vi "CIF_Iceoryx Channel Performance Test.vi"() -> ()   [LabVIEW 2021]
uses:
  Double/CIF_Iceoryx_Chn_Double.lvclass
  D:/dev/Packages/CIF_Channels_Core/src/Iceorxy_Channels/CIF_Iceoryx_BB/CIF_Iceoryx_BB.lvclass
  D:/dev/Packages/CIF_Channels_Core/src/CIFChannels/CIFChannels.lvclass
  ChannelCommon/typedef/Direction.ctl
  <vilib>/CIF Foundation/CIF Iceoryx/typedef/Topic Full Names.ctl
  <vilib>/Platform/TimedLoop/XDataNode/timing_clust.ctl
  <vilib>/Platform/TimedLoop/XDataNode/nitl_modes.ctl
  <vilib>/Platform/TimedLoop/XDataNode/wakeup.ctl
  ChannelCommon/typedef/New FIFO Instance Response.ctl
  CIFChannels/CIFChannels.lvclass/CIFChannels.ctl
  CIF_Iceoryx_BB/CIF_Iceoryx_BB.lvclass/CIF_Iceoryx_BB.ctl
  Double/CIF_Iceoryx_Chn_Double.lvclass/CIF_Iceoryx_Chn_Double.ctl
  53e91fa4-a651-41f7-b02c-832fa8f08f6c.vi
  a00a81b1-57b6-4108-a755-745f4eb81d77.vi
  b62546a3-05e7-4285-b37f-cb0405f50769.vi
  14a2fe34-1335-4f7a-a7a9-124bb301578e.vi
  14bdf759-0034-46fe-882d-46e8766a29d9.vi
  ec66e212-9a84-4060-a812-2933347e74f4.vi
  182f4b0c-1596-45c4-9e4a-6a0b9b3960fd.vi
  <vilib>/CIF Foundation/CIF Iceoryx/SubVIs/Get Path.vi
  <vilib>/CIF Foundation/CIF Iceoryx/SubVIs/Convert Error.vi
  53e91fa4-a651-41f7-b02c-832fa8f08f6c.vi/f164bb55-fadc-406a-97d8-e3295a396b46.vi
  <vilib>/CIF Foundation/CIF Iceoryx/SubVIs/Add Error.vi
  <vilib>/CIF Foundation/CIF Iceoryx/Refnum/BB from Refnum.vi
  <vilib>/CIF Foundation/CIF Iceoryx/Refnum/BB Writer to Refnum.vi
  a00a81b1-57b6-4108-a755-745f4eb81d77.vi/15451e88-64ef-462d-9cc0-58968935b893.vi
  <vilib>/CIF Foundation/CIF Iceoryx/Refnum/BB Writer from Refnum.vi
  <vilib>/CIF Foundation/CIF Iceoryx/Refnum/BB Reader from Refnum.vi
  Double/Core/Read Double Direct.vi/e9c5801a-3ed8-4028-afd6-45613173f8eb.vi
  CIF_Iceoryx_BB/Accessors/Read Reader Reference.vi
  CIFChannels/Accessors/Read Tag Forced.vi
  CIFChannels/Accessors/Read Channel State.vi
  CIFChannels/Accessors/Read Direction.vi
  Double/Core/Write Double Direct.vi/36393718-afdf-41a6-b430-da9823bc1f33.vi
  CIF_Iceoryx_BB/Accessors/Read Writer Reference.vi
  <vilib>/Utility/error.llb/Trim Whitespace.vi
  <vilib>/CIF Foundation/CIF Iceoryx/SubVIs/Add Error Core.vi
  <vilib>/CIF Foundation/CIF Utilities/DataTypes/Utilities/Get Element Info of Variant.vi
  <vilib>/CIF Foundation/CIF Iceoryx/SubVIs/Get Type String.vi
  <vilib>/CIF Foundation/CIF Utilities/DataTypes/Utilities/Get JSON Descriptor of Variant.vi
  <vilib>/CIF Foundation/CIF Iceoryx/SubVIs/Convert Error Core.vi
  <vilib>/CIF Foundation/CIF Iceoryx/Blackboard/Create Abstracted Reader.vi
  <vilib>/Platform/TimedLoop/XDataNode/XDataNode.xnode
  <vilib>/Platform/TimedLoop/XDataNode/XDNodeRunTimeDep.lvlib
  <vilib>/CIF Foundation/CIF Iceoryx/Iceoryx.lvlib
  ChannelCommon/ChannelCommon.lvlib
  CIF_Iceoryx_BB/CIF_Iceoryx_BB.lvclass
  CIFChannels/CIFChannels.lvclass
panel:
  out "avg dbl channel write":dbl
  out "max dbl channel write":dbl
  out "avg dbl channel dd":dbl
  out "max dbl channel dd":dbl
  in  "Stop":bool
  out "avg dbl channel":dbl
  out "max dbl channel":dbl
  out "avg raw channel":dbl
  out "max raw channel":dbl
  out "pass":bool
  out "error out":errorcluster
  # "This test should be run on RT.  It stresses the communications by constantly creating resource contraints with the low priority sender and the high priority loop. On Windows the priority of the loops cannot be set."
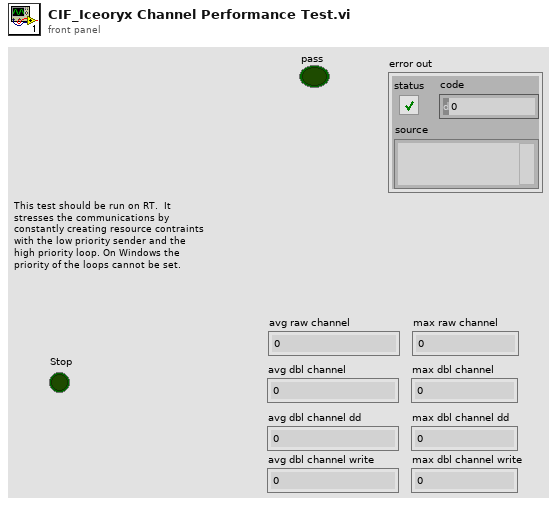
[diagram p1: front panel]
types:
  T1 = typedef "ChannelCommon.lvlib/Direction.ctl" = enum8{"Publisher", "Subscriber"}
  T2 = typedef "Iceoryx.lvlib/Topic Full Names.ctl" = cluster{"BlackBoard":string, "Topic":string, "Type Override":string}
  T3 = typedef "XDNodeRunTimeDep.lvlib/timing_clust.ctl" = cluster{"Expected End [f-1]":u64, "Actual End [f-1]":u64, "Finished Late? [f-1]":bool, "Expected End [i-1]":u64, "Actual End [i-1]":u64, "Finished Late? [i-1]":bool, "Expected Start [i]":u64, "Actual Start [i]":u64, "Expected Start [f]":u64, "Actual Start [f]":u64, "Source Name":string, "Structure Name":string, "Period":i64, "Deadline":i64, "Offset":i64, "Start":i64, "Priority":i32, "Timeout":i32, "Mode":T4, "Wakeup Reason":T5, "Error":errorcluster, "Source Type":string, "Secondary Source Type":string, "Global End Time":u64, "Global Start Time":u64, "Frame Duration":u64, "Iteration Duration":u64, "Assigned CPU":i32, "I/O Scan Engine Mode":u32}
  T4 = typedef "XDNodeRunTimeDep.lvlib/nitl_modes.ctl" = enum32{"No Change", "Process missed periods, maintain original phase", "Discard missed periods, maintain original phase", "Process missed periods, ignore original phase", "Discard missed periods, ignore original phase"}
  T5 = typedef "XDNodeRunTimeDep.lvlib/wakeup.ctl" = enum32{"Normal", "Aborted", "Asynchronous wakeup", "Timing source error", "Timed loop error", "Timeout"}
  T6 = typedef "ChannelCommon.lvlib/New FIFO Instance Response.ctl" = cluster{"Publisher":string, "Custom Data":u8[]}
  T7 = typedef "Iceoryx.lvlib/BB Refnum.ctl" = cluster{"refnum":u64, "BB":enum8{"bb"}}
  T8 = typedef "Iceoryx.lvlib/BB Writer Refnum.ctl" = cluster{"refnum":u64, "BB Writer":enum8{"bb_writer"}}
  T9 = typedef "Iceoryx.lvlib/BB Reader Refnum.ctl" = cluster{"refnum":u64, "BB Reader":enum8{"bb_reader"}}
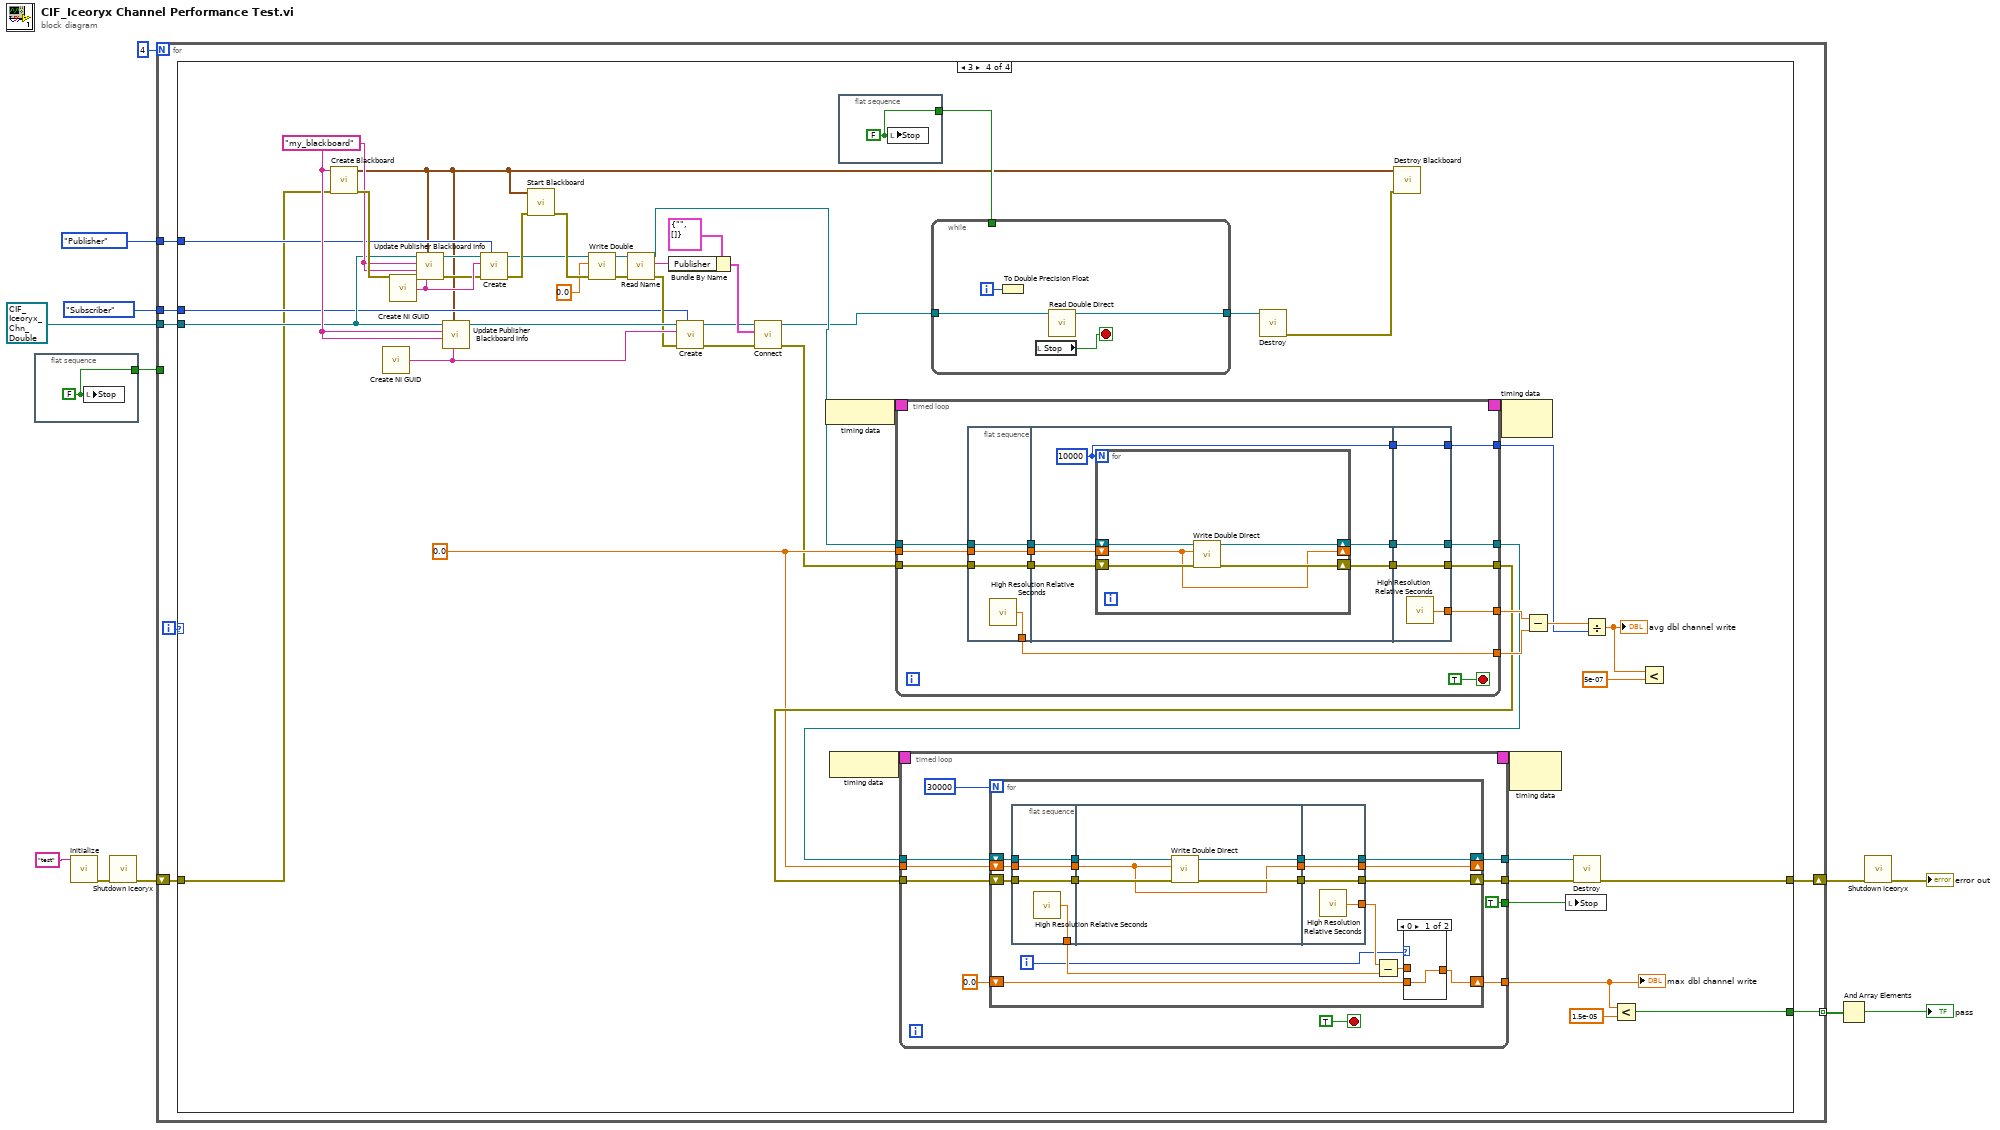
[diagram p0: block diagram]
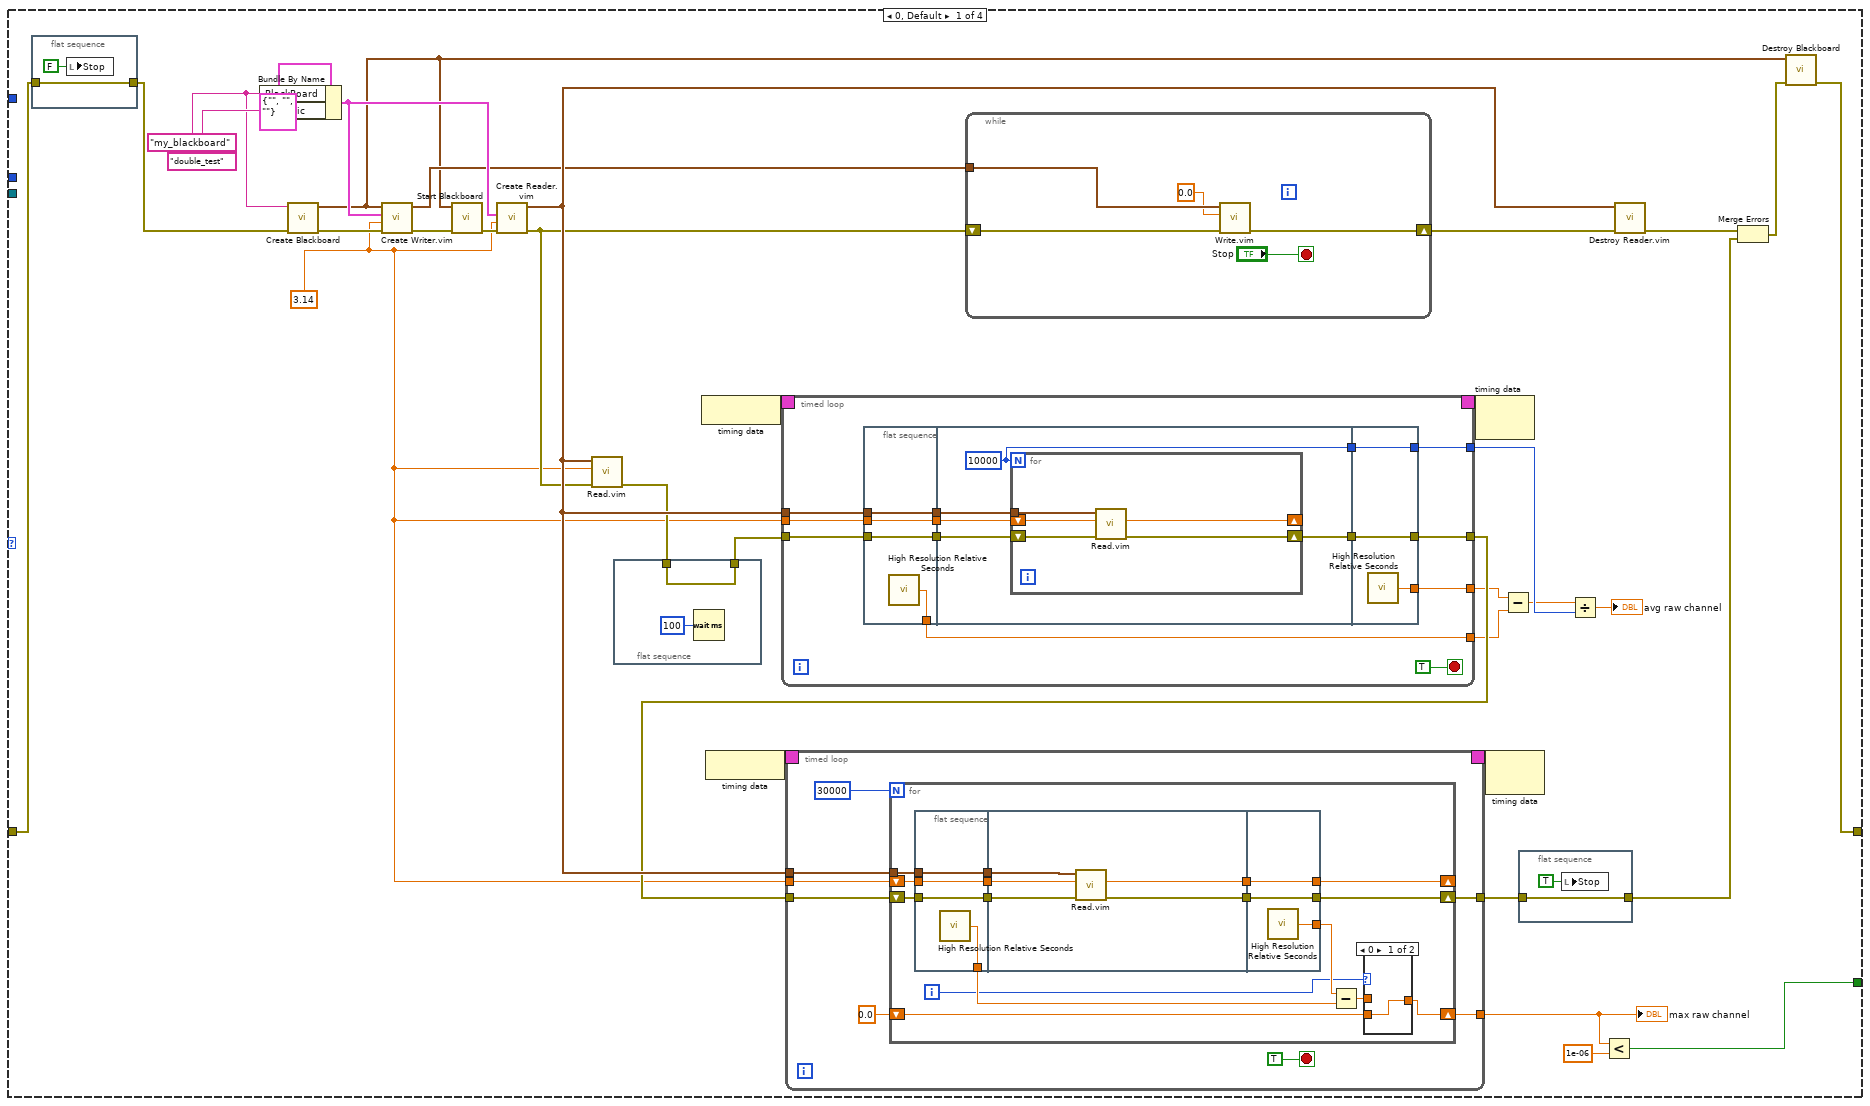
[diagram p2: hidden frame]
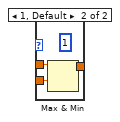
[diagram p3: hidden frame]
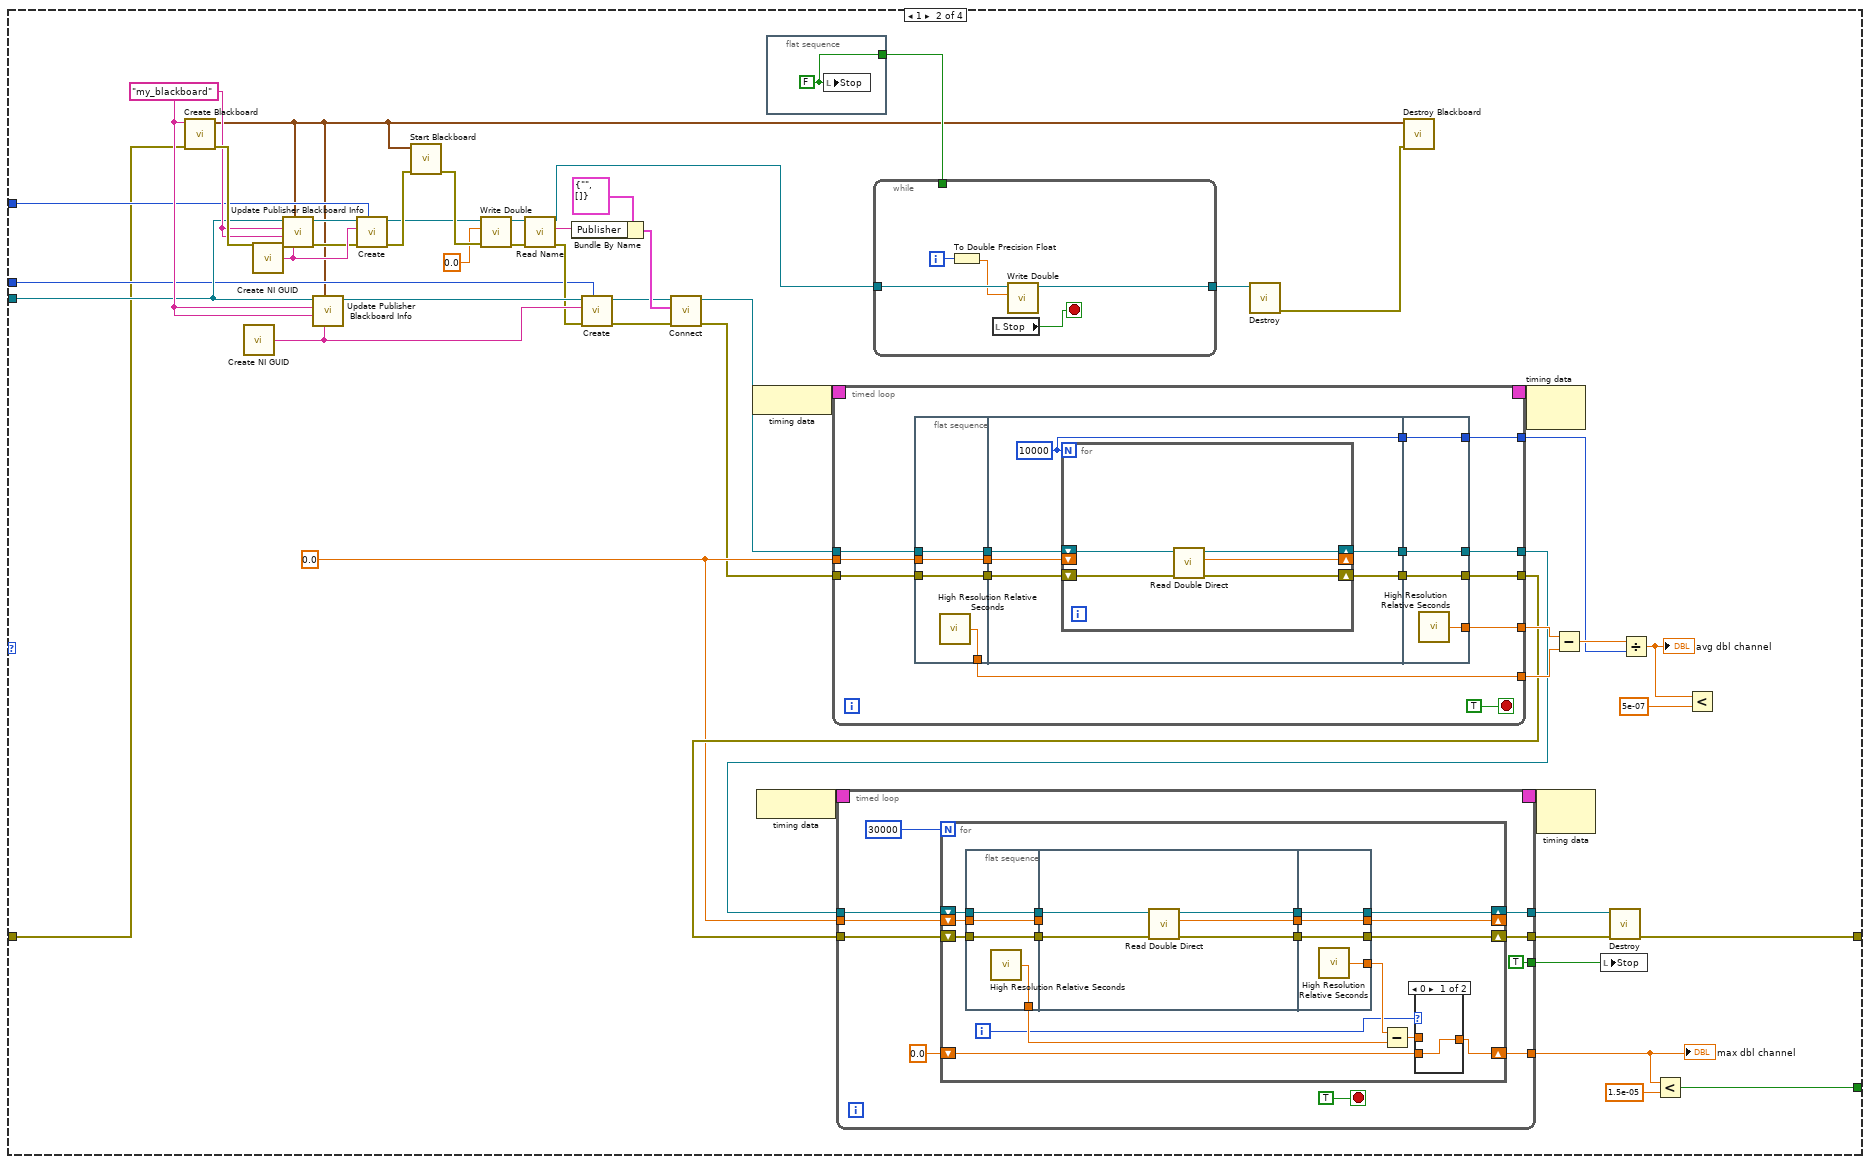
[diagram p4: hidden frame]
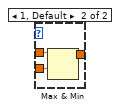
[diagram p5: hidden frame]
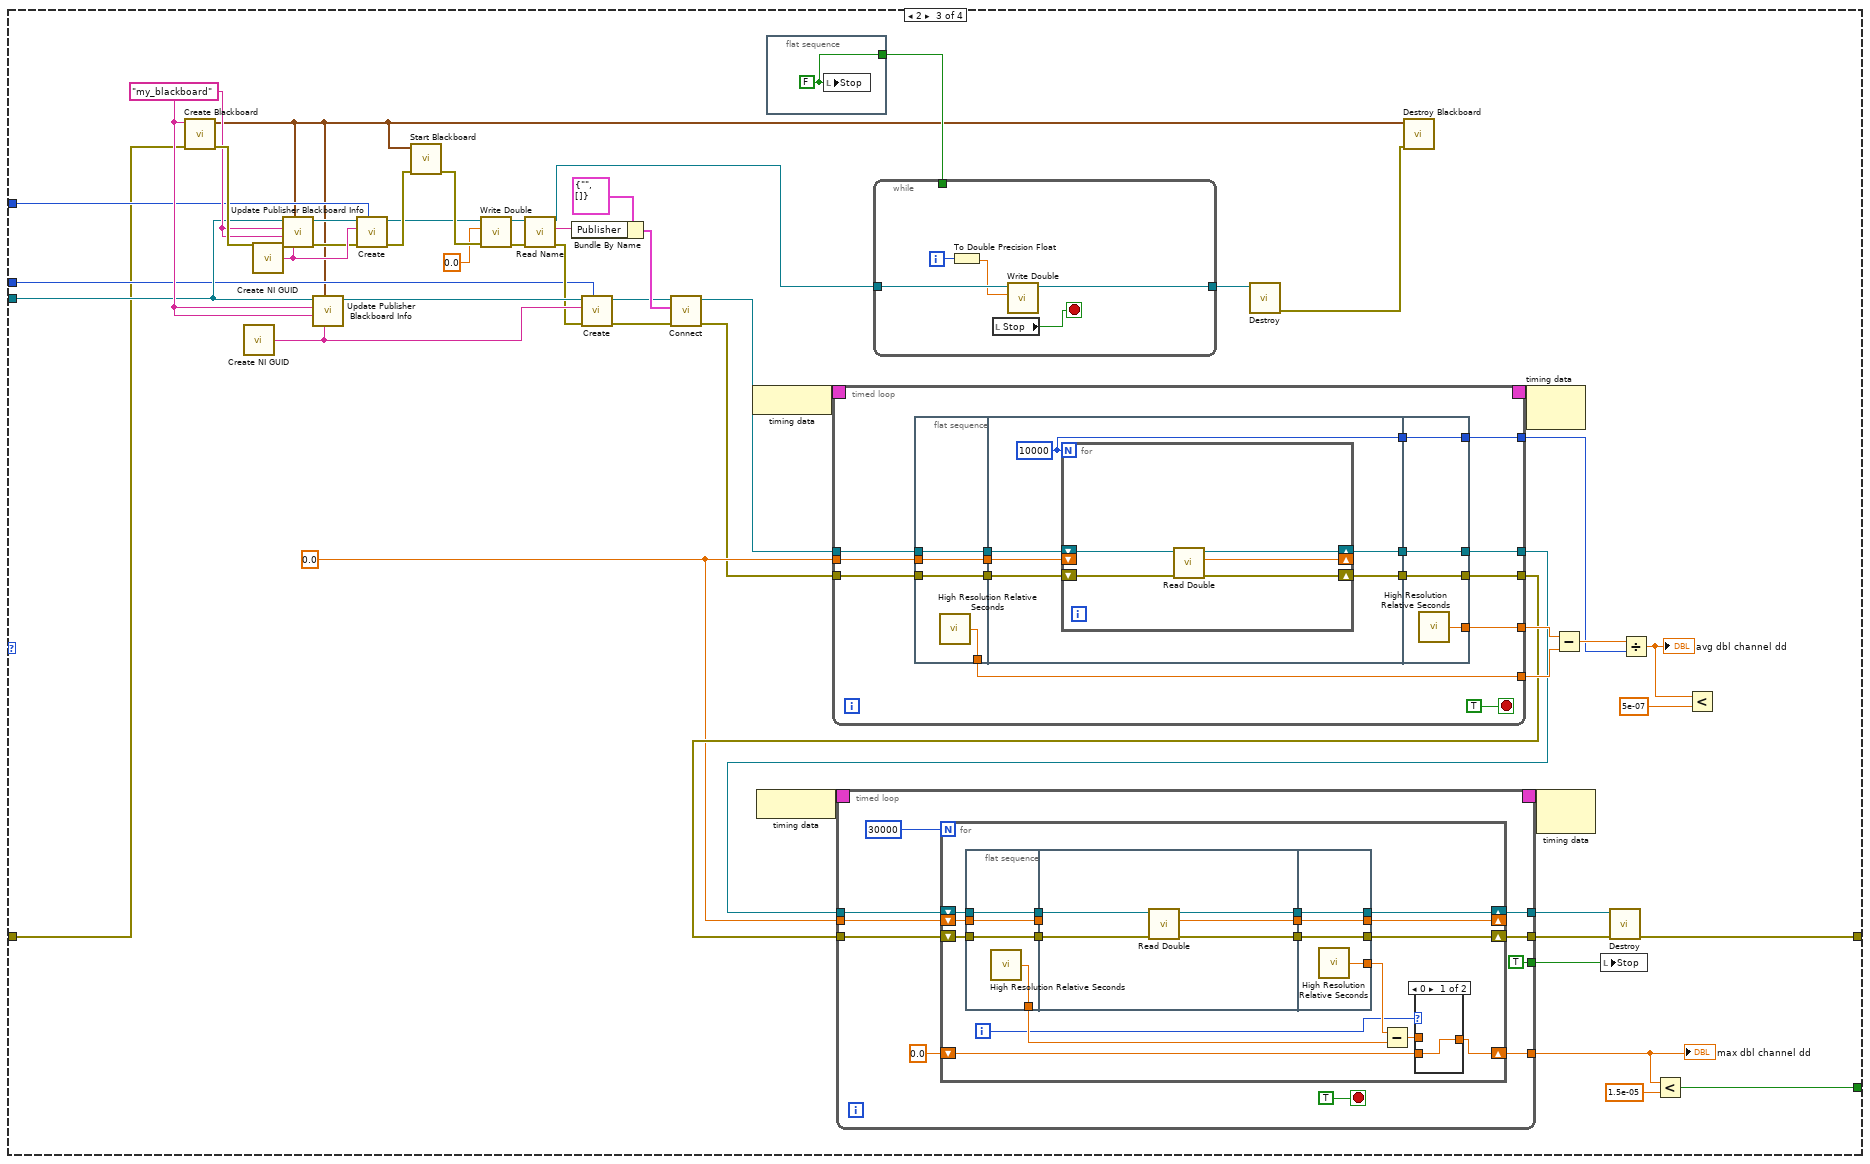
[diagram p6: hidden frame]
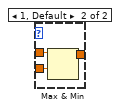
[diagram p7: hidden frame]
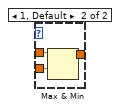
[diagram p8: hidden frame]
diagram:
  n1 = flat-sequence {
    tunnel: [w13] -> w8
    frame #0 {
      w13 = FALSE ("Stop")
      n2 = local write "Stop"(w13) -> ()
    }
  }
  n3 = call <vilib>:"Initialize.vi"("Node name"="test") -> ("error out"=w4:errorcluster)  [unwired: 10 in]
  n4 = call <vilib>:"Shutdown Iceoryx.vi"("error in (no error)"=w4) -> ("error out"=w3:errorcluster)  [unwired: 10 in]
  n5 = for {
    N: 4 -> [_]
    tunnel: [w20] -> w11 mode=indexing
    shift-right: [w19] -> w2
    shift-left: w3 -> [w17]
    tunnel: refnum<class "CIF_Iceoryx_Chn_Double.lvclass"> refnum ("CIF_CIPC_Chn_Double.lvclass") -> [w16]
    tunnel: w8 -> [_]
    tunnel: Direction."Publisher" ("Direction") -> [w15]
    tunnel: Direction."Subscriber" ("Direction") -> [w14]
    i -> [w18]
    n6 = case shown="3" w18 {
      tunnel: [w25 w180 w323 w466] -> w20
      tunnel: [w24 w176 w319 w462] -> w19
      tunnel: w17 -> [w30 w147 w290 w434]
      tunnel: w16 -> [_ w154 w297 w440]
      tunnel: w15 -> [_ w153 w296 w439]
      tunnel: w14 -> [_ w152 w295 w438]
      frame 0, Default {
        w22 = "my_blackboard" ("Blackboard name")
        w23 = 3.14 ("Data")
        n7 = flat-sequence {
          tunnel: w30 -> [w62]
          tunnel: [w62] -> w48
          frame #0 {
            n8 = local write "Stop"(FALSE ("stop")) -> ()
          }
        }
        n9 = Bundle By Name(cluster=T2 {"BlackBoard"="", "Topic"="", "Type Override"=""} ("Topic Full Names"), "BlackBoard"=w22, "Topic"="double_test" ("topic")) -> (w45:T2)
        n10 = call <vilib>:"Create Blackboard.vi"("error in (no error)"=w48, "Blackboard name"=w22) -> ("error out"=w38:errorcluster, "Blackboard Reference"=w40:T7)  [unwired: 8 in]
        n11 = call "Create Writer.vim"("error in (no error)"=w38, "Data"=w23, "Topic Name"=w45, "BlackBoard Reference"=w40) -> ("error out"=w39:errorcluster, "Writer Reference"=w42:T8)  [unwired: 5 in, 1 out]
        n12 = call <vilib>:"Start Blackboard.vi"("error in (no error)"=w39, "Blackboard Reference"=w40) -> ("error out"=w41:errorcluster)  [unwired: 9 in]
        n13 = call "Create Reader.vim"("error in (no error)"=w41, "Data Type"=w23, "Topic Name"=w45) -> ("error out"=w43:errorcluster, "Reader Reference"=w51:T9)  [unwired: 6 in, 1 out]
        n14 = call "Read.vim"("error in (no error)"=w43, "Data In"=w23, "Reader Reference"=w51) -> ("error out"=w44:errorcluster)  [unwired: 6 in, 2 out]
        n15 = flat-sequence {
          tunnel: w44 -> [w66]
          tunnel: [w66] -> w36
          frame #0 {
            n16 = Wait (ms)(milliseconds to wait=u32 100) -> ()  [unwired: 1 out]
          }
        }
        n17 = node-c288() -> (w55:T3)
        n18 = node-c288() -> (w53:T3)
        n19 = timed-loop {
          timing: w55 -> [_]
          timing-out: [_] -> w54
          tunnel: w51 -> [w113]
          tunnel: w36 -> [w123]
          tunnel: [w120] -> w35
          tunnel: [w118] -> w31
          tunnel: [w117] -> w32
          tunnel: [w116] -> w34
          tunnel: w23 -> [w111]
          stop <- TRUE stop-if-true
          n20 = flat-sequence {
            tunnel: w123 -> [w127]
            tunnel: [w127] -> w121
            tunnel: [w126] -> w117
            tunnel: [w125] -> w114
            tunnel: w113 -> [w125]
            tunnel: [w124] -> w112
            tunnel: w111 -> [w124]
            tunnel: w121 -> [w132]
            tunnel: [w131] -> w119
            tunnel: [w130] -> w115
            tunnel: w114 -> [w129]
            tunnel: w112 -> [w128]
            tunnel: [w140] -> w120
            tunnel: w119 -> [w140]
            tunnel: [w139] -> w118
            tunnel: [w138] -> w116
            tunnel: w115 -> [w138]
            frame #0 {
              n21 = call <vilib>:"High Resolution Relative Seconds.vi"() -> ("relative seconds"=w126:dbl)
            }
            frame #1 {
              w130 = 10000
              n22 = for {
                N: w130 -> [_]
                shift-right: [w134] -> _
                shift-left: w128 -> [w133]
                shift-right: [w135] -> w131
                shift-left: w132 -> [w136]
                tunnel: w129 -> [w137]
                n23 = call "Read.vim"("error in (no error)"=w136, "Data In"=w133, "Reader Reference"=w137) -> ("error out"=w135:errorcluster, "Data Out"=w134:dbl)  [unwired: 6 in, 1 out]
              }
            }
            frame #2 {
              n24 = call <vilib>:"High Resolution Relative Seconds.vi"() -> ("relative seconds"=w139:dbl)
            }
          }
        }
        n25 = timed-loop {
          timing: w53 -> [_]
          timing-out: [_] -> w52
          tunnel: w35 -> [w74]
          tunnel: [w72] -> w37
          tunnel: [w69] -> w26
          tunnel: w23 -> [w68]
          tunnel: w51 -> [w67]
          stop <- TRUE stop-if-true
          n26 = for {
            N: 30000 -> [_]
            shift-right: [w85] -> _
            shift-left: w68 -> [w87]
            shift-right: [w84] -> w72
            shift-left: w74 -> [w86]
            shift-right: [w79] -> w69
            shift-left: 0.0 -> [w80]
            tunnel: w67 -> [w75]
            i -> [w78]
            n27 = flat-sequence {
              tunnel: w86 -> [w97]
              tunnel: w87 -> [w98]
              tunnel: [w98] -> w90
              tunnel: [w97] -> w89
              tunnel: [w96] -> w82
              tunnel: [w95] -> w76
              tunnel: w75 -> [w95]
              tunnel: w90 -> [w99]
              tunnel: w89 -> [w103]
              tunnel: [w101] -> w88
              tunnel: [w100] -> w77
              tunnel: w76 -> [w102]
              tunnel: [w106] -> w85
              tunnel: w88 -> [w106]
              tunnel: [w105] -> w84
              tunnel: [w104] -> w83
              tunnel: w77 -> [w105]
              frame #0 {
                n28 = call <vilib>:"High Resolution Relative Seconds.vi"() -> ("relative seconds"=w96:dbl)
              }
              frame #1 {
                n29 = call "Read.vim"("error in (no error)"=w103, "Data In"=w99, "Reader Reference"=w102) -> ("error out"=w100:errorcluster, "Data Out"=w101:dbl)  [unwired: 6 in, 1 out]
              }
              frame #2 {
                n30 = call <vilib>:"High Resolution Relative Seconds.vi"() -> ("relative seconds"=w104:dbl)
              }
            }
            n31 = Subtract(x=w83, y=w82) -> (x-y=w81:dbl)
            n32 = case shown="0" w78 {
              tunnel: w81 -> [_ w94]
              tunnel: w80 -> [w91 w93]
              tunnel: [w91 w92] -> w79
              frame 0 {
              }
              frame 1, Default {
                (unwired) u32 1 ("milliseconds to wait")
                n33 = Max & Min(x=w94, y=w93) -> (max(x,y)=w92:dbl)  [unwired: 1 out]
              }
            }
          }
        }
        "max raw channel" <- w26
        n34 = while {
          shift-right: [w58] -> w49
          shift-left: w43 -> [w59]
          tunnel: w42 -> [w60]
          stop <- "Stop" stop-if-true
          n35 = call "Write.vim"("error in (no error)"=w59, "Data In"=0.0, "Writer Reference"=w60) -> ("error out"=w58:errorcluster)  [unwired: 7 in, 1 out]
        }
        n36 = node-c288(w54) -> ()  [unwired: 1 out]
        n37 = node-c288(w52) -> ()  [unwired: 1 out]
        n38 = Subtract(x=w31, y=w32) -> (x-y=w33:dbl)
        n39 = flat-sequence {
          tunnel: w37 -> [w64]
          tunnel: [w64] -> w46
          frame #0 {
            n40 = local write "Stop"(TRUE ("stop")) -> ()
          }
        }
        n41 = Divide(x=w33, y=w34) -> (x/y=→"avg raw channel":dbl)
        n42 = Less?(x=w26, y=1e-06) -> (x < y?=w25:bool)
        n43 = call "Destroy Reader.vim"("error in (no error)"=w49, "Reader Reference"=w51) -> ("error out"=w50:errorcluster)  [unwired: 9 in]
        n44 = Merge Errors(w50, w46) -> (w47:errorcluster)
        n45 = call <vilib>:"Destroy Blackboard.vi"("error in (no error)"=w47, "Blackboard Reference"=w40) -> ("error out"=w24:errorcluster)  [unwired: 8 in, 1 out]
      }
      frame 1 {
        w155 = "my_blackboard" ("Blackboard name")
        w177 = 0.0
        n46 = call <vilib>:"Create Blackboard.vi"("error in (no error)"=w147, "Blackboard name"=w155) -> ("error out"=w163:errorcluster, "Blackboard Reference"=w151:T7)  [unwired: 8 in]
        n47 = call <vilib>:"Create NI GUID.vi"() -> ("NI GUID"=w172:string)
        n48 = call <vilib>:"Create NI GUID.vi"() -> ("NI GUID"=w166:string)
        n49 = call "Update Publisher Blackboard Info.vi"("Topic"=w166, "Blackboard Reference"=w151, "error in (no error)"=w163, "Blackboard name"=w155, "Plugin name"=w155, "CIF_Iceoryx_BB in"=w154) -> ("error out"=w164:errorcluster, "CIF_Iceoryx_BB out"=w165:refnum<class "CIF_Iceoryx_Chn_Double.lvclass">)  [unwired: 3 in, 1 out]
        n50 = call "Update Publisher Blackboard Info.vi"("Topic"=w172, "Blackboard Reference"=w151, "Blackboard name"=w155, "Plugin name"=w155, "CIF_Iceoryx_BB in"=w154) -> ("CIF_Iceoryx_BB out"=w171:refnum<class "CIF_Iceoryx_Chn_Double.lvclass">)  [unwired: 4 in, 2 out]
        n51 = call-dynamic "Create.vi"("Direction"=w153, "error in (no error)"=w164, "Name"=w166, "CIF_Iceoryx_BB in"=w165) -> ("error out"=w161:errorcluster, "CIF_Iceoryx_BB out"=w159:refnum<class "CIF_Iceoryx_Chn_Double.lvclass">)  [unwired: 6 in]
        n52 = call <vilib>:"Start Blackboard.vi"("error in (no error)"=w161, "Blackboard Reference"=w151) -> ("error out"=w162:errorcluster)  [unwired: 9 in]
        n53 = call-dynamic "Write Double.vi"("error in (no error)"=w162, "Data"=0.0, "CIFTag in"=w159) -> ("error out"=w167:errorcluster, "CIFTag out"=w168:refnum<class "CIF_Iceoryx_Chn_Double.lvclass">)  [unwired: 6 in, 1 out]
        n54 = call "Read Name.vi"("error in (no error)"=w167, "CIFChannels in"=w168) -> ("error out"=w170:errorcluster, "Name"=w169:string, "CIFChannels out"=w149:refnum<class "CIF_Iceoryx_Chn_Double.lvclass">)  [unwired: 7 in]
        n55 = Bundle By Name(cluster=T6 {"Publisher"="", "Custom Data"=[]} ("Connection"), "Publisher"=w169) -> (w160:T6)
        n56 = call-dynamic "Create.vi"("Direction"=w152, "error in (no error)"=w170, "Name"=w172, "CIF_Iceoryx_BB in"=w171) -> ("error out"=w158:errorcluster, "CIF_Iceoryx_BB out"=w157:refnum<class "CIF_Iceoryx_Chn_Double.lvclass">)  [unwired: 6 in]
        n57 = call-dynamic "Connect.vi"("error in (no error)"=w158, "Connection"=w160, "CIF_Iceoryx_BB"=w157) -> ("error out"=w148:errorcluster, "CIF_Iceoryx_BB"=w145:refnum<class "CIF_Iceoryx_Chn_Double.lvclass">)  [unwired: 7 in]
        n58 = node-c288() -> (w194:T3)
        n59 = node-c288() -> (w192:T3)
        n60 = flat-sequence {
          tunnel: [w195] -> w174
          frame #0 {
            w195 = FALSE ("Stop")
            n61 = local write "Stop"(w195) -> ()
          }
        }
        n62 = timed-loop {
          timing: w194 -> [_]
          timing-out: [_] -> w193
          tunnel: w145 -> [w264]
          tunnel: w148 -> [w263]
          tunnel: [w259] -> w186
          tunnel: [w257] -> w185
          tunnel: [w255] -> w190
          tunnel: [w254] -> w189
          tunnel: [w253] -> w187
          tunnel: w177 -> [w251]
          stop <- TRUE stop-if-true
          n63 = flat-sequence {
            tunnel: w263 -> [w267]
            tunnel: w264 -> [w268]
            tunnel: [w268] -> w261
            tunnel: [w267] -> w260
            tunnel: [w266] -> w254
            tunnel: w251 -> [w265]
            tunnel: [w265] -> w250
            tunnel: w261 -> [w274]
            tunnel: w260 -> [w273]
            tunnel: [w272] -> w258
            tunnel: [w271] -> w256
            tunnel: [w270] -> w252
            tunnel: w250 -> [w269]
            tunnel: [w283] -> w259
            tunnel: w258 -> [w283]
            tunnel: [w282] -> w257
            tunnel: w256 -> [w282]
            tunnel: [w281] -> w255
            tunnel: [w280] -> w253
            tunnel: w252 -> [w280]
            frame #0 {
              n64 = call <vilib>:"High Resolution Relative Seconds.vi"() -> ("relative seconds"=w266:dbl)
            }
            frame #1 {
              w270 = 10000
              n65 = for {
                N: w270 -> [_]
                shift-right: [w276] -> w272
                shift-left: w274 -> [w279]
                shift-right: [w277] -> w271
                shift-left: w273 -> [w278]
                shift-right: [w275] -> _
                shift-left: w269 -> [_]
                n66 = call "Read Double Direct.vi"("error in (no error)"=w278, "CIFTag in"=w279) -> ("error out"=w277:errorcluster, "Data"=w275:dbl, "CIFTag out"=w276:refnum<class "CIF_Iceoryx_Chn_Double.lvclass">)  [unwired: 7 in]
              }
            }
            frame #2 {
              n67 = call <vilib>:"High Resolution Relative Seconds.vi"() -> ("relative seconds"=w281:dbl)
            }
          }
        }
        n68 = timed-loop {
          timing: w192 -> [_]
          timing-out: [_] -> w191
          tunnel: w186 -> [w210]
          tunnel: w185 -> [w209]
          tunnel: [w207] -> w178
          tunnel: [w206] -> w179
          tunnel: w177 -> [w205]
          tunnel: [w202] -> w182
          tunnel: [TRUE ("Stop")] -> w173
          stop <- TRUE stop-if-true
          n69 = for {
            N: 30000 -> [_]
            shift-right: [w222] -> w207
            shift-left: w210 -> [w224]
            shift-right: [w221] -> w206
            shift-left: w209 -> [w223]
            shift-right: [w215] -> w202
            shift-left: 0.0 -> [w216]
            shift-right: [w214] -> _
            shift-left: w205 -> [w220]
            i -> [w212]
            n70 = flat-sequence {
              tunnel: w223 -> [w235]
              tunnel: w224 -> [w236]
              tunnel: [w236] -> w228
              tunnel: [w235] -> w227
              tunnel: [w234] -> w218
              tunnel: w220 -> [w233]
              tunnel: [w233] -> w226
              tunnel: w228 -> [w241]
              tunnel: w227 -> [w238]
              tunnel: [w240] -> w225
              tunnel: w226 -> [_]
              tunnel: [w239] -> w213
              tunnel: [w237] -> w211
              tunnel: [w245] -> w222
              tunnel: w225 -> [w245]
              tunnel: [w244] -> w221
              tunnel: [w243] -> w219
              tunnel: [w242] -> w214
              tunnel: w213 -> [w242]
              tunnel: w211 -> [w244]
              frame #0 {
                n71 = call <vilib>:"High Resolution Relative Seconds.vi"() -> ("relative seconds"=w234:dbl)
              }
              frame #1 {
                n72 = call "Read Double Direct.vi"("error in (no error)"=w238, "CIFTag in"=w241) -> ("error out"=w237:errorcluster, "Data"=w239:dbl, "CIFTag out"=w240:refnum<class "CIF_Iceoryx_Chn_Double.lvclass">)  [unwired: 7 in]
              }
              frame #2 {
                n73 = call <vilib>:"High Resolution Relative Seconds.vi"() -> ("relative seconds"=w243:dbl)
              }
            }
            n74 = Subtract(x=w219, y=w218) -> (x-y=w217:dbl)
            n75 = case shown="0" w212 {
              tunnel: w217 -> [_ w232]
              tunnel: w216 -> [w229 w231]
              tunnel: [w229 w230] -> w215
              frame 0 {
              }
              frame 1, Default {
                n76 = Max & Min(x=w232, y=w231) -> (max(x,y)=w230:dbl)  [unwired: 1 out]
              }
            }
          }
        }
        "max dbl channel" <- w182
        n77 = while {
          tunnel: w149 -> [w199]
          tunnel: [w197] -> w175
          tunnel: w174 -> [_]
          i -> [w200]
          stop <- w196 stop-if-true
          n78 = To Double Precision Float(number=w200) -> (double precision float=w198:dbl)
          n79 = local read "Stop"() -> (w196:bool)
          n80 = call-dynamic "Write Double.vi"("Data"=w198, "CIFTag in"=w199) -> ("CIFTag out"=w197:refnum<class "CIF_Iceoryx_Chn_Double.lvclass">)  [unwired: 7 in, 2 out]
        }
        n81 = call-dynamic "Destroy.vi"("CIF_Iceoryx_BB in"=w175) -> ("error out"=w150:errorcluster)  [unwired: 9 in, 1 out]
        n82 = call <vilib>:"Destroy Blackboard.vi"("error in (no error)"=w150, "Blackboard Reference"=w151) -> ()  [unwired: 8 in, 2 out]
        n83 = node-c288(w193) -> ()  [unwired: 1 out]
        n84 = node-c288(w191) -> ()  [unwired: 1 out]
        n85 = Subtract(x=w190, y=w189) -> (x-y=w188:dbl)
        n86 = local write "Stop"(w173) -> ()
        n87 = call-dynamic "Destroy.vi"("error in (no error)"=w179, "CIF_Iceoryx_BB in"=w178) -> ("error out"=w176:errorcluster)  [unwired: 8 in, 1 out]
        n88 = Divide(x=w188, y=w187) -> (x/y=w184:dbl)
        "avg dbl channel" <- w184
        n89 = Less?(x=w182, y=1.5e-05) -> (x < y?=w180:bool)
        n90 = Less?(x=w184, y=5e-07) -> ()  [unwired: 1 out]
      }
      frame 2 {
        w298 = "my_blackboard" ("Blackboard name")
        w320 = 0.0
        n91 = call <vilib>:"Create Blackboard.vi"("error in (no error)"=w290, "Blackboard name"=w298) -> ("error out"=w306:errorcluster, "Blackboard Reference"=w294:T7)  [unwired: 8 in]
        n92 = call <vilib>:"Create NI GUID.vi"() -> ("NI GUID"=w315:string)
        n93 = call <vilib>:"Create NI GUID.vi"() -> ("NI GUID"=w309:string)
        n94 = call "Update Publisher Blackboard Info.vi"("Topic"=w309, "Blackboard Reference"=w294, "error in (no error)"=w306, "Blackboard name"=w298, "Plugin name"=w298, "CIF_Iceoryx_BB in"=w297) -> ("error out"=w307:errorcluster, "CIF_Iceoryx_BB out"=w308:refnum<class "CIF_Iceoryx_Chn_Double.lvclass">)  [unwired: 3 in, 1 out]
        n95 = call "Update Publisher Blackboard Info.vi"("Topic"=w315, "Blackboard Reference"=w294, "Blackboard name"=w298, "Plugin name"=w298, "CIF_Iceoryx_BB in"=w297) -> ("CIF_Iceoryx_BB out"=w314:refnum<class "CIF_Iceoryx_Chn_Double.lvclass">)  [unwired: 4 in, 2 out]
        n96 = call-dynamic "Create.vi"("Direction"=w296, "error in (no error)"=w307, "Name"=w309, "CIF_Iceoryx_BB in"=w308) -> ("error out"=w304:errorcluster, "CIF_Iceoryx_BB out"=w302:refnum<class "CIF_Iceoryx_Chn_Double.lvclass">)  [unwired: 6 in]
        n97 = call <vilib>:"Start Blackboard.vi"("error in (no error)"=w304, "Blackboard Reference"=w294) -> ("error out"=w305:errorcluster)  [unwired: 9 in]
        n98 = call-dynamic "Write Double.vi"("error in (no error)"=w305, "Data"=0.0, "CIFTag in"=w302) -> ("error out"=w310:errorcluster, "CIFTag out"=w311:refnum<class "CIF_Iceoryx_Chn_Double.lvclass">)  [unwired: 6 in, 1 out]
        n99 = call "Read Name.vi"("error in (no error)"=w310, "CIFChannels in"=w311) -> ("error out"=w313:errorcluster, "Name"=w312:string, "CIFChannels out"=w292:refnum<class "CIF_Iceoryx_Chn_Double.lvclass">)  [unwired: 7 in]
        n100 = Bundle By Name(cluster=T6 {"Publisher"="", "Custom Data"=[]} ("Connection"), "Publisher"=w312) -> (w303:T6)
        n101 = call-dynamic "Create.vi"("Direction"=w295, "error in (no error)"=w313, "Name"=w315, "CIF_Iceoryx_BB in"=w314) -> ("error out"=w301:errorcluster, "CIF_Iceoryx_BB out"=w300:refnum<class "CIF_Iceoryx_Chn_Double.lvclass">)  [unwired: 6 in]
        n102 = call-dynamic "Connect.vi"("error in (no error)"=w301, "Connection"=w303, "CIF_Iceoryx_BB"=w300) -> ("error out"=w291:errorcluster, "CIF_Iceoryx_BB"=w288:refnum<class "CIF_Iceoryx_Chn_Double.lvclass">)  [unwired: 7 in]
        n103 = node-c288() -> (w337:T3)
        n104 = node-c288() -> (w335:T3)
        n105 = flat-sequence {
          tunnel: [w338] -> w317
          frame #0 {
            w338 = FALSE ("Stop")
            n106 = local write "Stop"(w338) -> ()
          }
        }
        n107 = timed-loop {
          timing: w337 -> [_]
          timing-out: [_] -> w336
          tunnel: w288 -> [w407]
          tunnel: w291 -> [w406]
          tunnel: [w402] -> w329
          tunnel: [w400] -> w328
          tunnel: [w398] -> w333
          tunnel: [w397] -> w332
          tunnel: [w396] -> w330
          tunnel: w320 -> [w394]
          stop <- TRUE stop-if-true
          n108 = flat-sequence {
            tunnel: w406 -> [w410]
            tunnel: w407 -> [w411]
            tunnel: [w411] -> w404
            tunnel: [w410] -> w403
            tunnel: [w409] -> w397
            tunnel: w394 -> [w408]
            tunnel: [w408] -> w393
            tunnel: w404 -> [w417]
            tunnel: w403 -> [w416]
            tunnel: [w415] -> w401
            tunnel: [w414] -> w399
            tunnel: [w413] -> w395
            tunnel: w393 -> [w412]
            tunnel: [w426] -> w402
            tunnel: w401 -> [w426]
            tunnel: [w425] -> w400
            tunnel: w399 -> [w425]
            tunnel: [w424] -> w398
            tunnel: [w423] -> w396
            tunnel: w395 -> [w423]
            frame #0 {
              n109 = call <vilib>:"High Resolution Relative Seconds.vi"() -> ("relative seconds"=w409:dbl)
            }
            frame #1 {
              w413 = 10000
              n110 = for {
                N: w413 -> [_]
                shift-right: [w419] -> w415
                shift-left: w417 -> [w422]
                shift-right: [w420] -> w414
                shift-left: w416 -> [w421]
                shift-right: [w418] -> _
                shift-left: w412 -> [_]
                n111 = call-dynamic "Read Double.vi"("error in (no error)"=w421, "CIFTag in"=w422) -> ("error out"=w420:errorcluster, "Data"=w418:dbl, "CIFTag out"=w419:refnum<class "CIF_Iceoryx_Chn_Double.lvclass">)  [unwired: 6 in, 1 out]
              }
            }
            frame #2 {
              n112 = call <vilib>:"High Resolution Relative Seconds.vi"() -> ("relative seconds"=w424:dbl)
            }
          }
        }
        n113 = timed-loop {
          timing: w335 -> [_]
          timing-out: [_] -> w334
          tunnel: w329 -> [w353]
          tunnel: w328 -> [w352]
          tunnel: [w350] -> w321
          tunnel: [w349] -> w322
          tunnel: w320 -> [w348]
          tunnel: [w345] -> w325
          tunnel: [TRUE ("Stop")] -> w316
          stop <- TRUE stop-if-true
          n114 = for {
            N: 30000 -> [_]
            shift-right: [w365] -> w350
            shift-left: w353 -> [w367]
            shift-right: [w364] -> w349
            shift-left: w352 -> [w366]
            shift-right: [w358] -> w345
            shift-left: 0.0 -> [w359]
            shift-right: [w357] -> _
            shift-left: w348 -> [w363]
            i -> [w355]
            n115 = flat-sequence {
              tunnel: w366 -> [w378]
              tunnel: w367 -> [w379]
              tunnel: [w379] -> w371
              tunnel: [w378] -> w370
              tunnel: [w377] -> w361
              tunnel: w363 -> [w376]
              tunnel: [w376] -> w369
              tunnel: w371 -> [w384]
              tunnel: w370 -> [w381]
              tunnel: [w383] -> w368
              tunnel: w369 -> [_]
              tunnel: [w382] -> w356
              tunnel: [w380] -> w354
              tunnel: [w388] -> w365
              tunnel: w368 -> [w388]
              tunnel: [w387] -> w364
              tunnel: [w386] -> w362
              tunnel: [w385] -> w357
              tunnel: w356 -> [w385]
              tunnel: w354 -> [w387]
              frame #0 {
                n116 = call <vilib>:"High Resolution Relative Seconds.vi"() -> ("relative seconds"=w377:dbl)
              }
              frame #1 {
                n117 = call-dynamic "Read Double.vi"("error in (no error)"=w381, "CIFTag in"=w384) -> ("error out"=w380:errorcluster, "Data"=w382:dbl, "CIFTag out"=w383:refnum<class "CIF_Iceoryx_Chn_Double.lvclass">)  [unwired: 6 in, 1 out]
              }
              frame #2 {
                n118 = call <vilib>:"High Resolution Relative Seconds.vi"() -> ("relative seconds"=w386:dbl)
              }
            }
            n119 = Subtract(x=w362, y=w361) -> (x-y=w360:dbl)
            n120 = case shown="0" w355 {
              tunnel: w360 -> [_ w375]
              tunnel: w359 -> [w372 w374]
              tunnel: [w372 w373] -> w358
              frame 0 {
              }
              frame 1, Default {
                n121 = Max & Min(x=w375, y=w374) -> (max(x,y)=w373:dbl)  [unwired: 1 out]
              }
            }
          }
        }
        "max dbl channel dd" <- w325
        n122 = while {
          tunnel: w292 -> [w342]
          tunnel: [w340] -> w318
          tunnel: w317 -> [_]
          i -> [w343]
          stop <- w339 stop-if-true
          n123 = To Double Precision Float(number=w343) -> (double precision float=w341:dbl)
          n124 = local read "Stop"() -> (w339:bool)
          n125 = call-dynamic "Write Double.vi"("Data"=w341, "CIFTag in"=w342) -> ("CIFTag out"=w340:refnum<class "CIF_Iceoryx_Chn_Double.lvclass">)  [unwired: 7 in, 2 out]
        }
        n126 = call-dynamic "Destroy.vi"("CIF_Iceoryx_BB in"=w318) -> ("error out"=w293:errorcluster)  [unwired: 9 in, 1 out]
        n127 = call <vilib>:"Destroy Blackboard.vi"("error in (no error)"=w293, "Blackboard Reference"=w294) -> ()  [unwired: 8 in, 2 out]
        n128 = node-c288(w336) -> ()  [unwired: 1 out]
        n129 = node-c288(w334) -> ()  [unwired: 1 out]
        n130 = Subtract(x=w333, y=w332) -> (x-y=w331:dbl)
        n131 = local write "Stop"(w316) -> ()
        n132 = call-dynamic "Destroy.vi"("error in (no error)"=w322, "CIF_Iceoryx_BB in"=w321) -> ("error out"=w319:errorcluster)  [unwired: 8 in, 1 out]
        n133 = Divide(x=w331, y=w330) -> (x/y=w327:dbl)
        "avg dbl channel dd" <- w327
        n134 = Less?(x=w325, y=1.5e-05) -> (x < y?=w323:bool)
        n135 = Less?(x=w327, y=5e-07) -> ()  [unwired: 1 out]
      }
      frame 3 {
        w441 = "my_blackboard" ("Blackboard name")
        w463 = 0.0
        n136 = call <vilib>:"Create Blackboard.vi"("error in (no error)"=w434, "Blackboard name"=w441) -> ("error out"=w449:errorcluster, "Blackboard Reference"=w437:T7)  [unwired: 8 in]
        n137 = call <vilib>:"Create NI GUID.vi"() -> ("NI GUID"=w458:string)
        n138 = call <vilib>:"Create NI GUID.vi"() -> ("NI GUID"=w452:string)
        n139 = call "Update Publisher Blackboard Info.vi"("Topic"=w452, "Blackboard Reference"=w437, "error in (no error)"=w449, "Blackboard name"=w441, "Plugin name"=w441, "CIF_Iceoryx_BB in"=w440) -> ("error out"=w450:errorcluster, "CIF_Iceoryx_BB out"=w451:refnum<class "CIF_Iceoryx_Chn_Double.lvclass">)  [unwired: 3 in, 1 out]
        n140 = call "Update Publisher Blackboard Info.vi"("Topic"=w458, "Blackboard Reference"=w437, "Blackboard name"=w441, "Plugin name"=w441, "CIF_Iceoryx_BB in"=w440) -> ("CIF_Iceoryx_BB out"=w457:refnum<class "CIF_Iceoryx_Chn_Double.lvclass">)  [unwired: 4 in, 2 out]
        n141 = call-dynamic "Create.vi"("Direction"=w439, "error in (no error)"=w450, "Name"=w452, "CIF_Iceoryx_BB in"=w451) -> ("error out"=w447:errorcluster, "CIF_Iceoryx_BB out"=w445:refnum<class "CIF_Iceoryx_Chn_Double.lvclass">)  [unwired: 6 in]
        n142 = call <vilib>:"Start Blackboard.vi"("error in (no error)"=w447, "Blackboard Reference"=w437) -> ("error out"=w448:errorcluster)  [unwired: 9 in]
        n143 = call-dynamic "Write Double.vi"("error in (no error)"=w448, "Data"=0.0, "CIFTag in"=w445) -> ("error out"=w453:errorcluster, "CIFTag out"=w454:refnum<class "CIF_Iceoryx_Chn_Double.lvclass">)  [unwired: 6 in, 1 out]
        n144 = call "Read Name.vi"("error in (no error)"=w453, "CIFChannels in"=w454) -> ("error out"=w456:errorcluster, "Name"=w455:string, "CIFChannels out"=w432:refnum<class "CIF_Iceoryx_Chn_Double.lvclass">)  [unwired: 7 in]
        n145 = Bundle By Name(cluster=T6 {"Publisher"="", "Custom Data"=[]} ("Connection"), "Publisher"=w455) -> (w446:T6)
        n146 = call-dynamic "Create.vi"("Direction"=w438, "error in (no error)"=w456, "Name"=w458, "CIF_Iceoryx_BB in"=w457) -> ("error out"=w444:errorcluster, "CIF_Iceoryx_BB out"=w443:refnum<class "CIF_Iceoryx_Chn_Double.lvclass">)  [unwired: 6 in]
        n147 = call-dynamic "Connect.vi"("error in (no error)"=w444, "Connection"=w446, "CIF_Iceoryx_BB"=w443) -> ("error out"=w435:errorcluster, "CIF_Iceoryx_BB"=w431:refnum<class "CIF_Iceoryx_Chn_Double.lvclass">)  [unwired: 7 in]
        n148 = node-c288() -> (w480:T3)
        n149 = node-c288() -> (w478:T3)
        n150 = flat-sequence {
          tunnel: [w481] -> w460
          frame #0 {
            w481 = FALSE ("Stop")
            n151 = local write "Stop"(w481) -> ()
          }
        }
        n152 = timed-loop {
          timing: w480 -> [_]
          timing-out: [_] -> w479
          tunnel: w432 -> [w549]
          tunnel: w435 -> [w548]
          tunnel: [w544] -> w472
          tunnel: [w542] -> w471
          tunnel: [w540] -> w476
          tunnel: [w539] -> w475
          tunnel: [w538] -> w473
          tunnel: w463 -> [w536]
          stop <- TRUE stop-if-true
          n153 = flat-sequence {
            tunnel: w548 -> [w552]
            tunnel: w549 -> [w553]
            tunnel: [w553] -> w546
            tunnel: [w552] -> w545
            tunnel: [w551] -> w539
            tunnel: w536 -> [w550]
            tunnel: [w550] -> w535
            tunnel: w546 -> [w559]
            tunnel: w545 -> [w558]
            tunnel: [w557] -> w543
            tunnel: [w556] -> w541
            tunnel: [w555] -> w537
            tunnel: w535 -> [w554]
            tunnel: [w568] -> w544
            tunnel: w543 -> [w568]
            tunnel: [w567] -> w542
            tunnel: w541 -> [w567]
            tunnel: [w566] -> w540
            tunnel: [w565] -> w538
            tunnel: w537 -> [w565]
            frame #0 {
              n154 = call <vilib>:"High Resolution Relative Seconds.vi"() -> ("relative seconds"=w551:dbl)
            }
            frame #1 {
              w555 = 10000
              n155 = for {
                N: w555 -> [_]
                shift-right: [w561] -> w557
                shift-left: w559 -> [w564]
                shift-right: [w562] -> w556
                shift-left: w558 -> [w563]
                shift-right: [w560] -> _
                shift-left: w554 -> [w560]
                n156 = call "Write Double Direct.vi"("error in (no error)"=w563, "Data"=w560, "CIFTag in"=w564) -> ("error out"=w562:errorcluster, "CIFTag out"=w561:refnum<class "CIF_Iceoryx_Chn_Double.lvclass">)  [unwired: 7 in]
              }
            }
            frame #2 {
              n157 = call <vilib>:"High Resolution Relative Seconds.vi"() -> ("relative seconds"=w566:dbl)
            }
          }
        }
        n158 = timed-loop {
          timing: w478 -> [_]
          timing-out: [_] -> w477
          tunnel: w472 -> [w495]
          tunnel: w471 -> [w494]
          tunnel: [w492] -> w464
          tunnel: [w491] -> w465
          tunnel: w463 -> [w490]
          tunnel: [w487] -> w468
          tunnel: [TRUE ("Stop")] -> w459
          stop <- TRUE stop-if-true
          n159 = for {
            N: 30000 -> [_]
            shift-right: [w507] -> w492
            shift-left: w495 -> [w509]
            shift-right: [w506] -> w491
            shift-left: w494 -> [w508]
            shift-right: [w500] -> w487
            shift-left: 0.0 -> [w501]
            shift-right: [w499] -> _
            shift-left: w490 -> [w505]
            i -> [w497]
            n160 = flat-sequence {
              tunnel: w508 -> [w520]
              tunnel: w509 -> [w521]
              tunnel: [w521] -> w513
              tunnel: [w520] -> w512
              tunnel: [w519] -> w503
              tunnel: w505 -> [w518]
              tunnel: [w518] -> w511
              tunnel: w513 -> [w526]
              tunnel: w512 -> [w524]
              tunnel: [w525] -> w510
              tunnel: w511 -> [w522]
              tunnel: [w522] -> w498
              tunnel: [w523] -> w496
              tunnel: [w530] -> w507
              tunnel: w510 -> [w530]
              tunnel: [w529] -> w506
              tunnel: [w528] -> w504
              tunnel: [w527] -> w499
              tunnel: w498 -> [w527]
              tunnel: w496 -> [w529]
              frame #0 {
                n161 = call <vilib>:"High Resolution Relative Seconds.vi"() -> ("relative seconds"=w519:dbl)
              }
              frame #1 {
                n162 = call "Write Double Direct.vi"("error in (no error)"=w524, "Data"=w522, "CIFTag in"=w526) -> ("error out"=w523:errorcluster, "CIFTag out"=w525:refnum<class "CIF_Iceoryx_Chn_Double.lvclass">)  [unwired: 7 in]
              }
              frame #2 {
                n163 = call <vilib>:"High Resolution Relative Seconds.vi"() -> ("relative seconds"=w528:dbl)
              }
            }
            n164 = Subtract(x=w504, y=w503) -> (x-y=w502:dbl)
            n165 = case shown="0" w497 {
              tunnel: w502 -> [_ w517]
              tunnel: w501 -> [w514 w516]
              tunnel: [w514 w515] -> w500
              frame 0 {
              }
              frame 1, Default {
                n166 = Max & Min(x=w517, y=w516) -> (max(x,y)=w515:dbl)  [unwired: 1 out]
              }
            }
          }
        }
        "max dbl channel write" <- w468
        n167 = while {
          tunnel: w431 -> [w484]
          tunnel: [w483] -> w461
          tunnel: w460 -> [_]
          i -> [w485]
          stop <- w482 stop-if-true
          n168 = To Double Precision Float(number=w485) -> ()  [unwired: 1 out]
          n169 = local read "Stop"() -> (w482:bool)
          n170 = call "Read Double Direct.vi"("CIFTag in"=w484) -> ("CIFTag out"=w483:refnum<class "CIF_Iceoryx_Chn_Double.lvclass">)  [unwired: 8 in, 2 out]
        }
        n171 = call-dynamic "Destroy.vi"("CIF_Iceoryx_BB in"=w461) -> ("error out"=w436:errorcluster)  [unwired: 9 in, 1 out]
        n172 = call <vilib>:"Destroy Blackboard.vi"("error in (no error)"=w436, "Blackboard Reference"=w437) -> ()  [unwired: 8 in, 2 out]
        n173 = node-c288(w479) -> ()  [unwired: 1 out]
        n174 = node-c288(w477) -> ()  [unwired: 1 out]
        n175 = Subtract(x=w476, y=w475) -> (x-y=w474:dbl)
        n176 = local write "Stop"(w459) -> ()
        n177 = call-dynamic "Destroy.vi"("error in (no error)"=w465, "CIF_Iceoryx_BB in"=w464) -> ("error out"=w462:errorcluster)  [unwired: 8 in, 1 out]
        n178 = Divide(x=w474, y=w473) -> (x/y=w470:dbl)
        "avg dbl channel write" <- w470
        n179 = Less?(x=w468, y=1.5e-05) -> (x < y?=w466:bool)
        n180 = Less?(x=w470, y=5e-07) -> ()  [unwired: 1 out]
      }
    }
  }
  n181 = And Array Elements(Boolean array=w11) -> (logical AND=→"pass":bool)
  n182 = call <vilib>:"Shutdown Iceoryx.vi"("error in (no error)"=w2) -> ("error out"=→"error out":errorcluster)  [unwired: 10 in]
